vi "R_Path.vi"(8 "error in (no error)":errorcluster caption="错误输入（无错误）", 11 "Path_management输入":refnum<class "Path_management.lvclass">) -> (0 "error out":errorcluster caption="错误输出", 2 "Path":path[](array[path]), 3 "Path_management输出":refnum<class "Path_management.lvclass">)   [LabVIEW 2025, in "Path_management.lvclass"]
uses:
  Path_management.lvclass
  Path_management.lvclass/Path_management.ctl
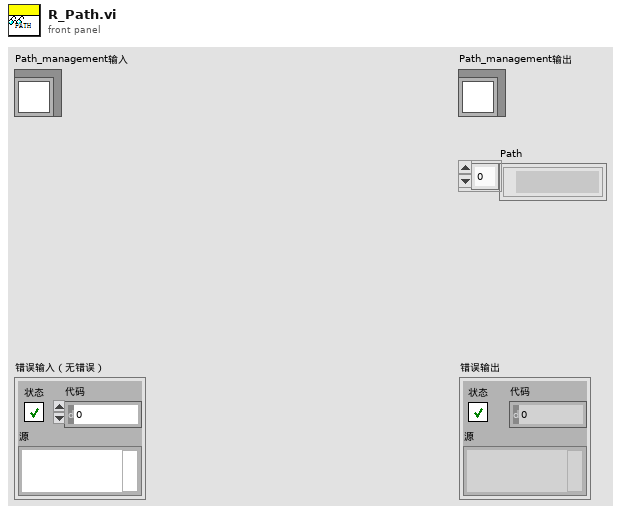
[diagram p1: front panel]
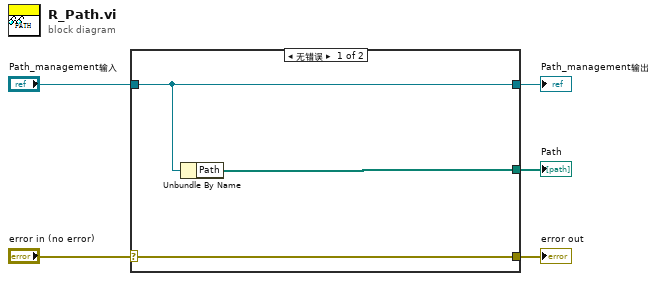
[diagram p0: block diagram]
diagram:
  n1 = case shown="无错误" "error in (no error)" {
    selector: "error in (no error)" -> [w8 w9]
    tunnel: [w8 w9] -> w4
    tunnel: [w7 w10] -> w2
    tunnel: "Path_management输入" -> [w7 w10]
    tunnel: [w6 _] -> w1
    frame No Error {
      n2 = Unbundle By Name(w7) -> ("Path"=w6:path[])
    }
    frame Error {
    }
  }
  "error out" <- w4
  "Path_management输出" <- w2
  "Path" <- w1
